vi "Resample Data.vi"(10 "dt":dbl, 11 "Data Series In":T1[](array[typedef])) -> (3 "Data Series Out":T1[](array[typedef]))   [LabVIEW 2020, in "Data Viewer.lvlib" / "Data Viewer.lvclass"]
uses:
  Data Viewer.lvclass
  Data Serie--cluster.ctl
  <vilib>/measure/maresamp.llb/Resample Waveform (single shot).vi
  <vilib>/measure/NI_MAPro.lvlib
  Data Viewer.lvlib
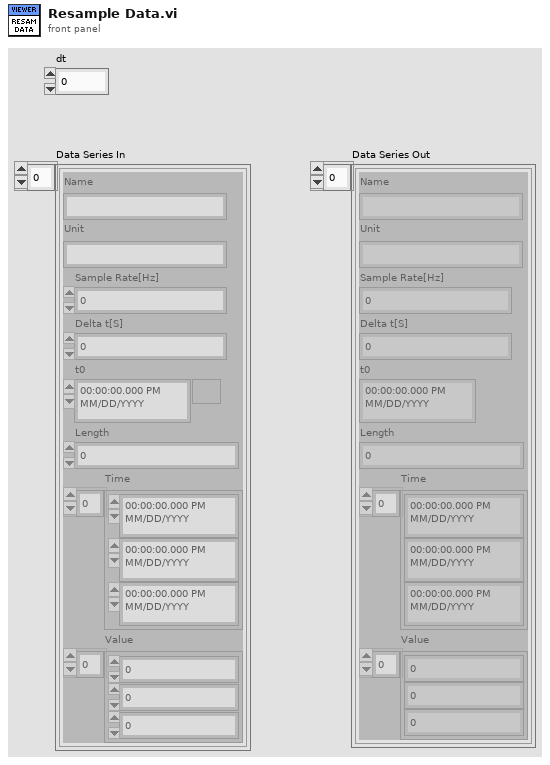
[diagram p1: front panel]
types:
  T1 = typedef "Data Viewer.lvlib/Data Serie--cluster.ctl" = cluster{"Name":string, "Unit":string, "Sample Rate[Hz]":dbl, "Delta t[S]":dbl, "t0":timestamp, "Length":i32, "Time":timestamp[], "Value":dbl[]}
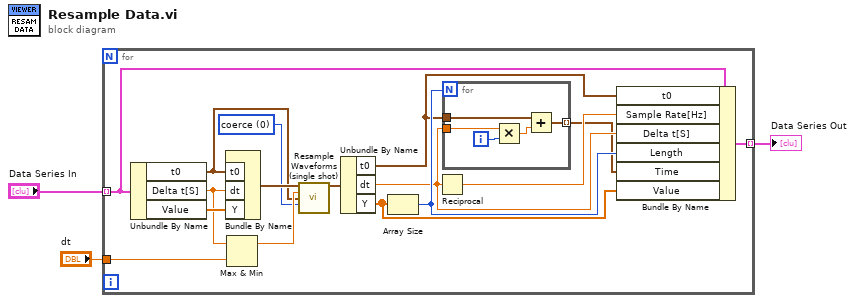
[diagram p0: block diagram]
diagram:
  n1 = for {
    tunnel: "Data Series In" -> [w11] mode=indexing
    tunnel: "dt" -> [w16]
    tunnel: [w8] -> w1 mode=indexing
    w13 = u16 0 items=["coerce", "linear", "spline", "FIR filter"] ("interpolation mode")
    n2 = Unbundle By Name(w11) -> ("t0"=w14:timestamp, "Delta t[S]"=w17:dbl, "Value"=w19:dbl[])
    n3 = Bundle By Name("t0"=w14, "dt"=w17, "Y"=w19) -> (w18:waveform(dbl))  [unwired: 1 in]
    n4 = Max & Min(x=w17, y=w16) -> (max(x,y)=w15:dbl)  [unwired: 1 out]
    n5 = call-poly <vilib>:"Resample Waveforms (single shot).vi"("waveform in"=w18, "dt"=w15, "t0"=w14, "interpolation mode"=w13) -> ("resampled waveform out"=w12:waveform(dbl))  [unwired: 8 in, 3 out]
    n6 = Unbundle By Name(w12) -> ("t0"=w6:timestamp, "dt"=w5:dbl, "Y"=w9:dbl[])
    n7 = Array Size(array=w9) -> (size(s)=w7:i32)
    n8 = Reciprocal(x=w5) -> (1/x=w10:dbl)
    n9 = for {
      N: w7 -> [_]
      tunnel: w6 -> [w24]
      tunnel: w5 -> [w21]
      tunnel: [w20] -> w4 mode=indexing
      i -> [w23]
      n10 = Multiply(x=w21, y=w23) -> (x*y=w22:dbl)
      n11 = Add(x=w24, y=w22) -> (x+y=w20:timestamp)
    }
    n12 = Bundle By Name(cluster=w11, "t0"=w6, "Sample Rate[Hz]"=w10, "Delta t[S]"=w5, "Length"=w7, "Time"=w4, "Value"=w9) -> (w8:T1)
  }
  "Data Series Out" <- w1
